vi "Edit Entry Dialog.vi"(8 "error in":errorcluster, 9 "Insert Mode? (F)":bool, 10 "Time Entry":T1, 11 "Project Store in":refnum<class "Project Store.lvclass">) -> (0 "error out":errorcluster, 1 "Updated?":bool, 2 "Edited Entry":T1, 3 "Project Store out":refnum<class "Project Store.lvclass">)   [LabVIEW 2026]
doc: "Dialog for editing one time entry: its project, task, start time, end time and description - or, with Insert Mode? (F) TRUE, for inserting a new entry inside it.\n\nOn open, Project lists the active projects (Project List.vi) and Task the active tasks of the entry's project (Task List.vi), both with the entry's own project and task selected. If the entry's project or task has since been made inactive, it is added to the end of its list so that it stays selected (Find or Add List Item.vi). Changing Project reloads Task with that project's tasks and selects the first one.\n\nEdit mode (Insert Mode? (F) FALSE, the default): a running entry (End Time = 0) keeps running: End Time is greyed out and is saved as 0. OK checks that a task is selected and, for a stopped entry, that End Time is not before Start Time. Edited Entry is the entry with the new values (same ID).\n\nInsert mode (Insert Mode? (F) TRUE): Time Entry is the ORIGINAL entry. The window title reads Insert Time Entry and the Original indicator shows the original's project / task and its start - end times (or running); it is hidden in Edit mode. Project and Task start at the original's; Start Time and End Time start as a 15-minute slot centred in the original (for a running original, centred between its start and now; the whole entry when it is shorter than 15 minutes); End Time is editable even for a running original; Description starts empty. OK checks that a task is selected, that Start Time is not before the original's Start Time, that End Time is not after the original's End Time (not after now for a running original) and that End Time is after Start Time. Edited Entry is the INSERTED entry: empty ID, the chosen Project ID and Task ID, Start Time, End Time and Description. The caller splits the original with Insert Entry.vi.\n\nIn both modes a failed check shows a message and keeps the dialog open; a valid OK gives Updated? TRUE. OK and Cancel are switch-when-pressed buttons that the dialog resets on open (and OK after a failed check), so they can also be pressed through Value (Signaling). Cancel returns Time Entry unchanged with Updated? FALSE. Nothing is written to disk here: the caller saves Edited Entry.\n\nInputs: Project Store in; Time Entry; Insert Mode? (F); error in.\nOutputs: Project Store out; Edited Entry; Updated?; error out.\n\nGenerated by: Claude"
uses:
  Storage/Project Store/Project Store.lvclass
  Storage/Rows/Time Entry.ctl
panel:
  out "Original":string
  in  "Cancel":bool
  in  "OK":bool
  in  "Project":u16(ring)
  in  "Task":u16(ring)
  in  "Start Time":timestamp
  in  "End Time":timestamp
  in  "Description":string
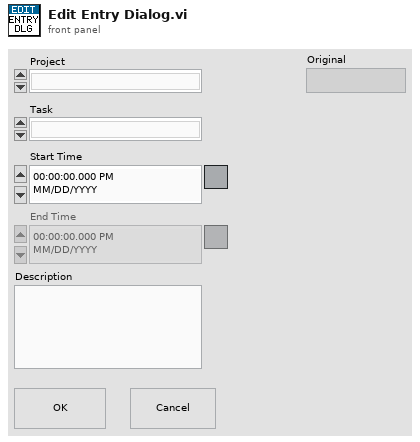
[diagram p1: front panel]
types:
  T1 = typedef "Time Entry.ctl" = cluster{"ID":string, "Project ID":string, "Task ID":string, "Start Time":timestamp, "End Time":timestamp, "Description":string}
  T2 = typedef "Project.ctl" = cluster{"ID":string, "Name":string, "Active":bool, "Sort Order":i32}
  T3 = typedef "Task.ctl" = cluster{"ID":string, "Project ID":string, "Name":string, "Active":bool, "Sort Order":i32}
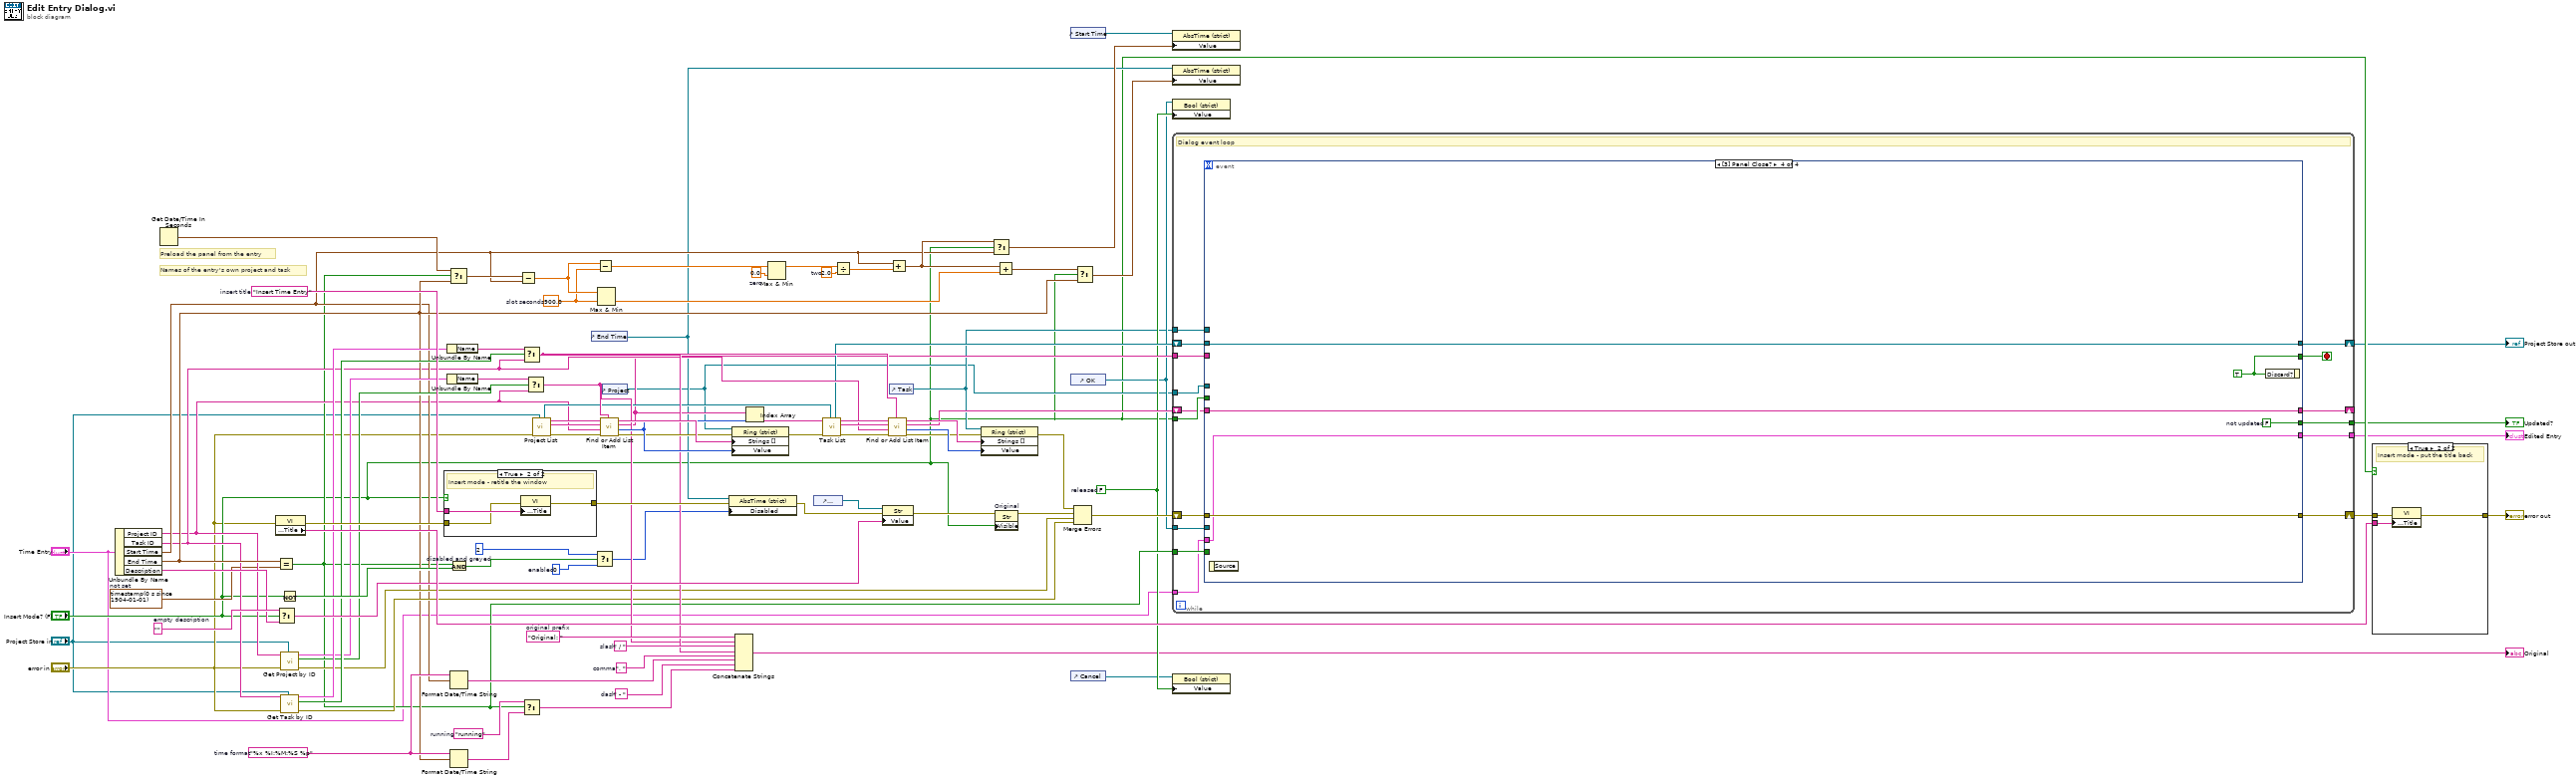
[diagram p0: block diagram]
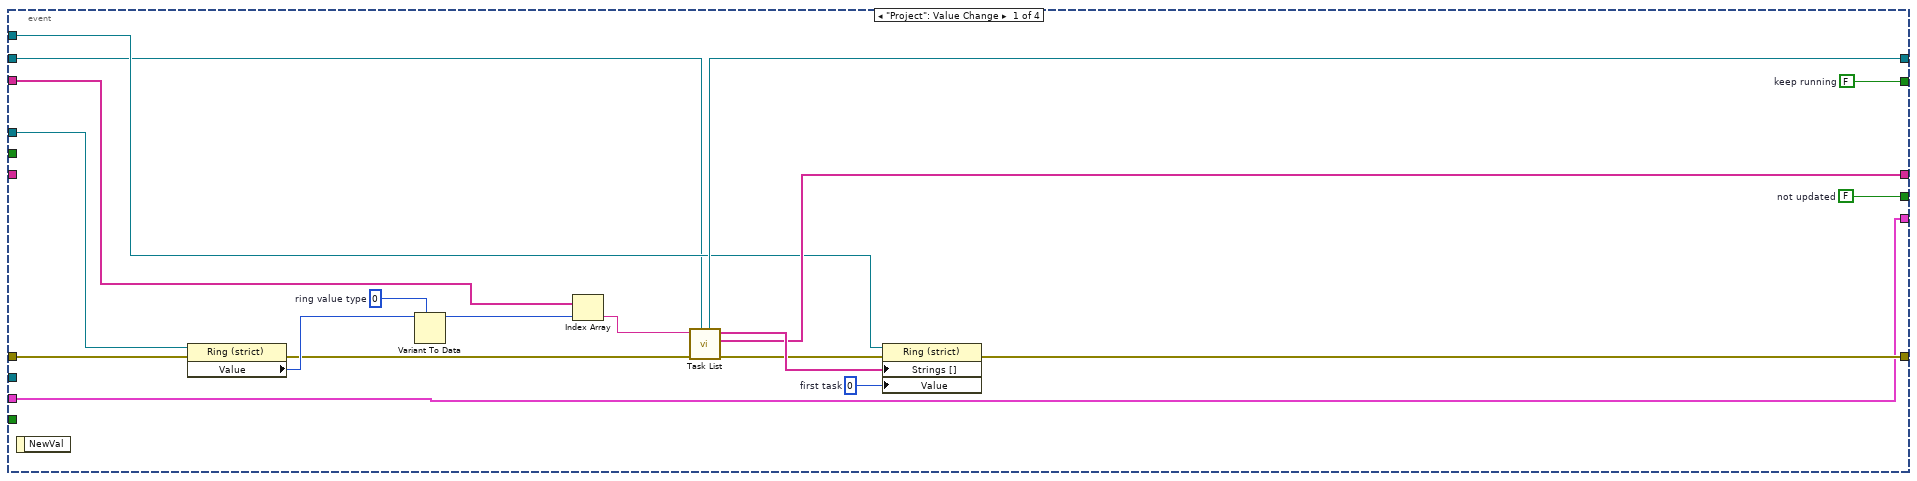
[diagram p4: hidden frame]
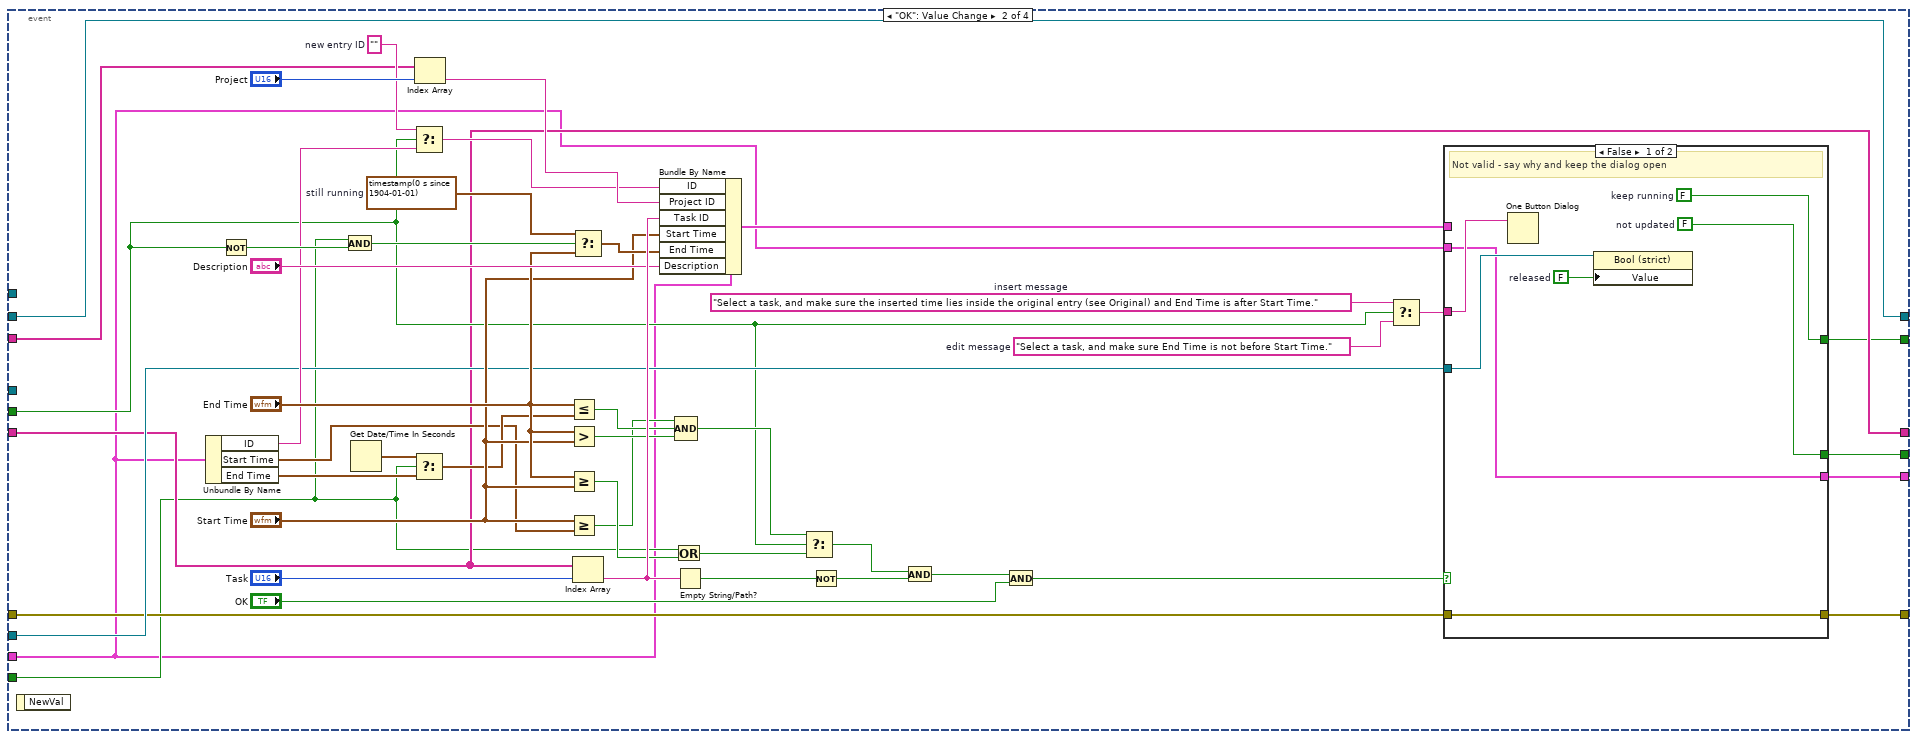
[diagram p5: hidden frame]
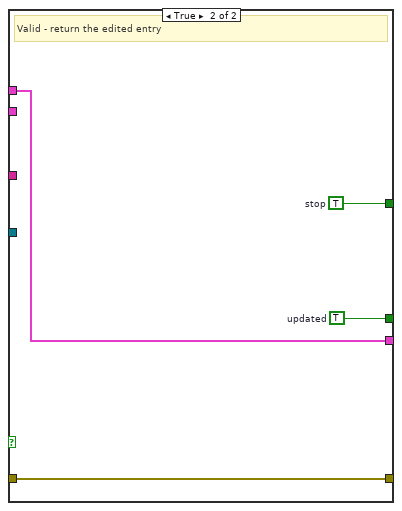
[diagram p6: hidden frame]
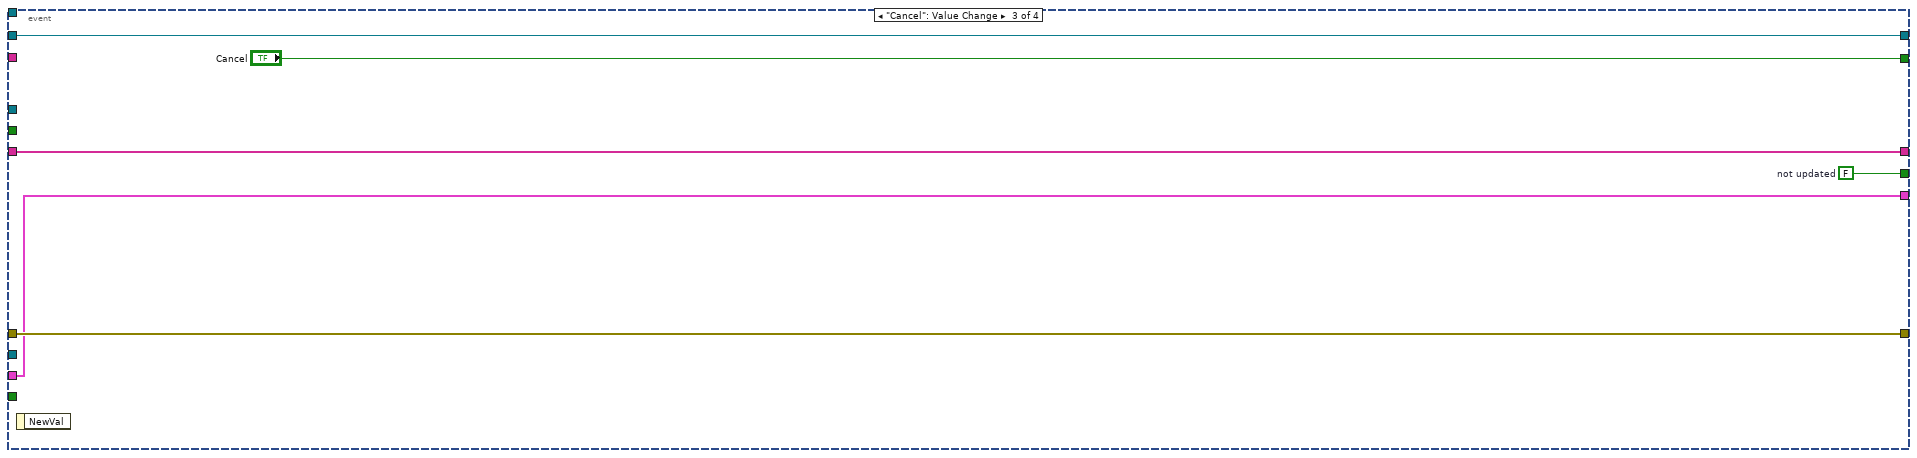
[diagram p7: hidden frame]
diagram:
  w92 = "Insert Time Entry"  # insert title
  w86 = "Original: "  # original prefix
  w85 = " - "  # dash
  w84 = ", "  # comma
  w83 = " / "  # slash
  w82 = "running"  # running
  w81 = "%x %I:%M:%S %p"  # time format
  w71 = ""  # empty description
  w70 = 2.0  # two
  w69 = 0.0  # zero
  w68 = 900.0  # slot seconds
  w20 = u8 0  # enabled
  w19 = u8 2  # disabled and greyed
  w18 = timestamp(0 s since 1904-01-01)  # not set
  w17 = FALSE  # released
  # "Names of the entry's own project and task"
  # "Preload the panel from the entry"
  n1 = Unbundle By Name("Time Entry") -> ("Project ID"=w27:string, "Task ID"=w28:string, "Start Time"=w29:timestamp, "End Time"=w30:timestamp, "Description"=w31:string)
  n2 = Get Date/Time In Seconds() -> (seconds since 1Jan1904=w67:timestamp)
  n3 = property class="VI"(error in="error in") -> (error out=w90:errorcluster, "Front Panel Window:Title"=w91:string)  [unwired: 1 in, 1 out]
  n4 = Equal?(x=w30, y=w18) -> (x = y?=w21:bool)
  n5 = Select(t=w71, s="Insert Mode? (F)", f=w31) -> (s? t:f=w56:string)
  n6 = Not(x="Insert Mode? (F)") -> (.not. x?=w80:bool)
  n7 = call-dynamic "Get Project by ID.vi"("Project Store in"="Project Store in", "error in (no error)"="error in", "ID"=w27) -> ("error out"=w36:errorcluster, "found?"=w37:bool, "Project"=w38:T2)  [unwired: 5 in, 1 out]
  n8 = call-dynamic "Get Task by ID.vi"("Project Store in"="Project Store in", "error in (no error)"="error in", "ID"=w28) -> ("error out"=w39:errorcluster, "found?"=w40:bool, "Task"=w41:T3)  [unwired: 5 in, 1 out]
  n9 = case shown="True" "Insert Mode? (F)" {
    tunnel: w92 -> [_ w95]
    tunnel: w90 -> [w93 w94]
    tunnel: [w93 w96] -> w51
    frame False {
    }
    frame True {
      # "Insert mode - retitle the window"
      n10 = property class="VI"(error in=w94, "Front Panel Window:Title"=w95) -> (error out=w96:errorcluster)  [unwired: 1 in, 1 out]
    }
  }
  n11 = Unbundle By Name(w41) -> ("Name"=w45:string)
  n12 = Unbundle By Name(w38) -> ("Name"=w44:string)
  n13 = Select(t=w67, s=w21, f=w30) -> (s? t:f=w72:timestamp)
  n14 = And(x=w21, y=w80) -> (x .and. y?=w47:bool)
  n15 = Format Date/Time String(time format string (%c)=w81, seconds (now)=w29) -> (date/time string=w87:string)  [unwired: 1 out]
  n16 = Format Date/Time String(time format string (%c)=w81, seconds (now)=w30) -> (date/time string=w88:string)  [unwired: 1 out]
  n17 = Subtract(x=w72, y=w29) -> (x-y=w73:dbl)
  n18 = Select(t=w45, s=w40, f=w28) -> (s? t:f=w49:string)
  n19 = Select(t=w82, s=w21, f=w88) -> (s? t:f=w89:string)
  n20 = Select(t=w44, s=w37, f=w27) -> (s? t:f=w48:string)
  n21 = call "Project List.vi"("Project Store in"="Project Store in", "error in"="error in") -> ("error out"=w32:errorcluster, "Project IDs"=w33:string[], "Project Names"=w34:string[], "Project Store out"=w35:refnum<class "Project Store.lvclass">)  [unwired: 6 in]
  n22 = control-ref of="End Time"() -> (w14:refnum<vi>)
  n23 = Select(t=w19, s=w47, f=w20) -> (s? t:f=w46:u8)
  n24 = Subtract(x=w73, y=w68) -> (x-y=w74:dbl)
  n25 = Max & Min(x=w73, y=w68) -> (min(x,y)=w77:dbl)  [unwired: 1 out]
  n26 = call "Find or Add List Item.vi"("Name"=w48, "error in"=w32, "ID"=w27, "IDs"=w33, "Names"=w34) -> ("error out"=w52:errorcluster, "Index"=w53:i32, "IDs out"=w22:string[], "Names out"=w54:string[])  [unwired: 3 in]
  n27 = control-ref of="Project"() -> (w10:refnum<vi>)
  n28 = property class="AbsTime (strict)"(reference=w14, error in=w51, "Disabled"=w46) -> (error out=w50:errorcluster)  [unwired: 1 out]
  n29 = property class="Ring (strict)"(reference=w10, error in=w52, "Strings []"=w54, "Value"=w53) -> (error out=w57:errorcluster)  [unwired: 1 out]
  n30 = Concatenate Strings(w86, w48, w83, w49, w84, w87, w85, w89) -> (→"Original":string)
  n31 = Index Array(array=w22, index=w53) -> (element=w58:string)
  n32 = Max & Min(x=w74, y=w69) -> (max(x,y)=w75:dbl)  [unwired: 1 out]
  n33 = control-ref of="Description"() -> (w12:refnum<vi>)
  n34 = call "Task List.vi"("Project Store in"=w35, "error in"=w57, "Project ID"=w58) -> ("error out"=w59:errorcluster, "Task IDs"=w60:string[], "Task Names"=w61:string[], "Project Store out"=w23:refnum<class "Project Store.lvclass">)  [unwired: 5 in]
  n35 = Divide(x=w75, y=w70) -> (x/y=w76:dbl)
  n36 = property class="Str"(reference=w12, error in=w50, "Value"=w56) -> (error out=w55:errorcluster)  [unwired: 1 out]
  n37 = call "Find or Add List Item.vi"("Name"=w49, "error in"=w59, "ID"=w28, "IDs"=w60, "Names"=w61) -> ("error out"=w62:errorcluster, "Index"=w63:i32, "IDs out"=w24:string[], "Names out"=w64:string[])  [unwired: 3 in]
  n38 = control-ref of="Task"() -> (w11:refnum<vi>)
  n39 = Add(x=w29, y=w76) -> (x+y=w78:timestamp)
  n40 = property class="Ring (strict)"(reference=w11, error in=w62, "Strings []"=w64, "Value"=w63) -> (error out=w65:errorcluster)  [unwired: 1 out]
  n41 = Select(t=w78, s="Insert Mode? (F)", f=w29) -> (s? t:f=w42:timestamp)
  n42 = property on="Original" class="Str"(error in=w55, "Visible"="Insert Mode? (F)") -> (error out=w66:errorcluster)  [unwired: 1 in, 1 out]
  n43 = Add(x=w78, y=w77) -> (x+y=w79:timestamp)
  n44 = control-ref of="Start Time"() -> (w13:refnum<vi>)
  n45 = control-ref of="OK"() -> (w15:refnum<vi>)
  n46 = control-ref of="Cancel"() -> (w16:refnum<vi>)
  n47 = Merge Errors(w65, w66, w36, w39) -> (w25:errorcluster)
  n48 = Select(t=w79, s="Insert Mode? (F)", f=w30) -> (s? t:f=w43:timestamp)
  n49 = property class="AbsTime (strict)"(reference=w13, "Value"=w42) -> ()  [unwired: 1 in, 2 out]
  n50 = property class="AbsTime (strict)"(reference=w14, "Value"=w43) -> ()  [unwired: 1 in, 2 out]
  n51 = property class="Bool (strict)"(reference=w15, "Value"=w17) -> ()  [unwired: 1 in, 2 out]
  n52 = while {
    tunnel: "Time Entry" -> [w97]
    tunnel: "Insert Mode? (F)" -> [w103]
    tunnel: w10 -> [w104]
    tunnel: w11 -> [w105]
    tunnel: w15 -> [w106]
    tunnel: [w108] -> w6
    tunnel: w21 -> [w98]
    tunnel: [w109] -> w5
    tunnel: w22 -> [w99]
    shift-right: [w111] -> w4
    shift-left: w23 -> [w100]
    shift-right: [w110] -> _
    shift-left: w24 -> [w101]
    shift-right: [w112] -> w26
    shift-left: w25 -> [w102]
    stop <- w107 stop-if-true
    # "Dialog event loop"
    n53 = event shown="[3] Panel Close?" {
      selector: _ -> [_ _ _ _]
      dyn-events: _ -> [_ _ _ _]
      timeout: _ -> [_ _ _ _]
      tunnel: [w113 w132 "Cancel" w195] -> w107
      tunnel: [w114 w133 w190 w196] -> w108
      tunnel: w97 -> [w115 w134 w191 w197]
      tunnel: w103 -> [_ w141 _ _]
      tunnel: w104 -> [w119 _ _ _]
      tunnel: w105 -> [w120 _ _ _]
      tunnel: w106 -> [_ w142 _ _]
      tunnel: [w115 w135 w191 w197] -> w109
      tunnel: w98 -> [_ w136 _ _]
      tunnel: w99 -> [w116 w137 _ _]
      tunnel: w100 -> [w117 w138 w192 w198]
      tunnel: w101 -> [_ w139 w193 w199]
      tunnel: w102 -> [w118 w140 w194 w200]
      tunnel: [w121 w139 w193 w199] -> w110
      tunnel: [w122 w138 w192 w198] -> w111
      tunnel: [w123 w163 w194 w200] -> w112
      event "Project": Value Change {
        w127 = u16 0  # ring value type
        w114 = FALSE  # not updated
        w113 = FALSE  # keep running
        w124 = u16 0  # first task
        n54 = event-data() -> ()  [unwired: 1 in, 1 out]
        n55 = property class="Ring (strict)"(reference=w119, error in=w118) -> (error out=w125:errorcluster, "Value"=w126:u16)  [unwired: 1 out]
        n56 = Variant To Data(type=w127, Variant=w126) -> (data=w128:u16)  [unwired: 1 in, 1 out]
        n57 = Index Array(array=w116, index=w128) -> (element=w129:string)
        n58 = call "Task List.vi"("Project Store in"=w117, "error in"=w125, "Project ID"=w129) -> ("error out"=w130:errorcluster, "Task IDs"=w121:string[], "Task Names"=w131:string[], "Project Store out"=w122:refnum<class "Project Store.lvclass">)  [unwired: 5 in]
        n59 = property class="Ring (strict)"(reference=w120, error in=w130, "Strings []"=w131, "Value"=w124) -> (error out=w123:errorcluster)  [unwired: 1 out]
      }
      event "OK": Value Change {
        w168 = timestamp(0 s since 1904-01-01)  # still running
        w161 = "Select a task, and make sure the inserted time lies inside the original entry (see Original) and End Time is after Start Time."  # insert message
        w160 = "Select a task, and make sure End Time is not before Start Time."  # edit message
        w158 = ""  # new entry ID
        n60 = event-data() -> ()  [unwired: 1 in, 1 out]
        n61 = Unbundle By Name(w134) -> ("ID"=w143:string, "Start Time"=w144:timestamp, "End Time"=w145:timestamp)
        n62 = Not(x=w141) -> (.not. x?=w156:bool)
        n63 = And(x=w136, y=w156) -> (x .and. y?=w157:bool)
        n64 = Get Date/Time In Seconds() -> (seconds since 1Jan1904=w146:timestamp)
        n65 = Select(t=w158, s=w141, f=w143) -> (s? t:f=w159:string)
        n66 = Select(t=w146, s=w136, f=w145) -> (s? t:f=w147:timestamp)
        n67 = Index Array(array=w137, index="Project") -> (element=w173:string)
        n68 = Less Or Equal?(x="End Time", y=w147) -> (x <= y?=w150:bool)
        n69 = Greater?(x="End Time", y="Start Time") -> (0:w152:bool)
        n70 = Greater Or Equal?(x="End Time", y="Start Time") -> (x >= y?=w171:bool)
        n71 = Greater Or Equal?(x="Start Time", y=w144) -> (x >= y?=w148:bool)
        n72 = Select(t=w168, s=w157, f="End Time") -> (s? t:f=w172:timestamp)
        n73 = Index Array(array=w139, index="Task") -> (element=w174:string)
        n74 = Bundle By Name(cluster=w134, "ID"=w159, "Project ID"=w173, "Task ID"=w174, "Start Time"="Start Time", "End Time"=w172, "Description"="Description") -> (w170:T1)
        n75 = Or(x=w136, y=w171) -> (x .or. y?=w155:bool)
        n76 = Compound Arithmetic op=AND(w148, w150, w152) -> (w153:bool)
        n77 = Empty String/Path?(string/path=w174) -> (empty?=w175:bool)
        n78 = Select(t=w153, s=w141, f=w155) -> (s? t:f=w154:bool)
        n79 = Not(x=w175) -> (.not. x?=w176:bool)
        n80 = And(x=w154, y=w176) -> (x .and. y?=w177:bool)
        n81 = And(x=w177, y="OK") -> (x .and. y?=w169:bool)
        n82 = Select(t=w161, s=w141, f=w160) -> (s? t:f=w162:string)
        n83 = case shown="False" w169 {
          tunnel: [w178 w185] -> w132
          tunnel: [w179 w186] -> w133
          tunnel: w134 -> [w180 _]
          tunnel: w142 -> [w183 _]
          tunnel: w162 -> [w182 _]
          tunnel: [w180 w187] -> w135
          tunnel: w170 -> [_ w187]
          tunnel: w140 -> [w181 w188]
          tunnel: [w181 w188] -> w163
          frame False {
            w179 = FALSE  # not updated
            w178 = FALSE  # keep running
            w184 = FALSE  # released
            # "Not valid - say why and keep the dialog open"
            n84 = One Button Dialog(message=w182) -> ()  [unwired: 1 in, 1 out]
            n85 = property class="Bool (strict)"(reference=w183, "Value"=w184) -> ()  [unwired: 1 in, 2 out]
          }
          frame True {
            w186 = TRUE  # updated
            w185 = TRUE  # stop
            # "Valid - return the edited entry"
          }
        }
      }
      event "Cancel": Value Change {
        w190 = FALSE  # not updated
        n86 = event-data() -> ()  [unwired: 1 in, 1 out]
      }
      event Panel Close? {
        w195 = TRUE ("Discard?")
        w196 = FALSE  # not updated
        n87 = event-data() -> ()  [unwired: 1 in, 1 out]
        n88 = event-data("Discard?"=w195) -> ()  [unwired: 1 in, 1 out]
      }
    }
  }
  "Project Store out" <- w4
  "Edited Entry" <- w5
  "Updated?" <- w6
  n89 = property class="Bool (strict)"(reference=w16, "Value"=w17) -> ()  [unwired: 1 in, 2 out]
  n90 = case shown="True" "Insert Mode? (F)" {
    tunnel: w91 -> [_ w203]
    tunnel: w26 -> [w201 w202]
    tunnel: [w201 w204] -> w7
    frame False {
    }
    frame True {
      # "Insert mode - put the title back"
      n91 = property class="VI"(error in=w202, "Front Panel Window:Title"=w203) -> (error out=w204:errorcluster)  [unwired: 1 in, 1 out]
    }
  }
  "error out" <- w7
